vi "电流捕捉 v2.vi"(0 "task/channels in":refnum<k21> caption="任务/通道输入", 1 "触发后延时":u32=50, 2 "驱动值":dbl=10.0 format="%#_13g", 5 "条件":dbl=1.0, 7 "停止次数":i32=10, 11 "采样数":i32=500, 12 "CurrentType":enum16{"RMS均方根值", "AVG平均值"}(ring), 13 "停止值":dbl=1.0 format="%#_13g") -> (3 "输出波形":waveform(dbl), 4 "task out":refnum<k21>, 6 "最大电流":dbl format="%0.2f", 8 "电流值":dbl caption="均方根值" format="%.4f", 10 "能量":dbl, 15 "持续时间":dbl format="%0.2f")   [LabVIEW 2025]
uses:
  global.vi
  <vilib>/DAQmx/miscellaneous.llb/DAQmx Fill In Error Info.vi
  <vilib>/measure/NI_MAPro.lvlib
  <vilib>/Analysis/NI_AALBase.lvlib
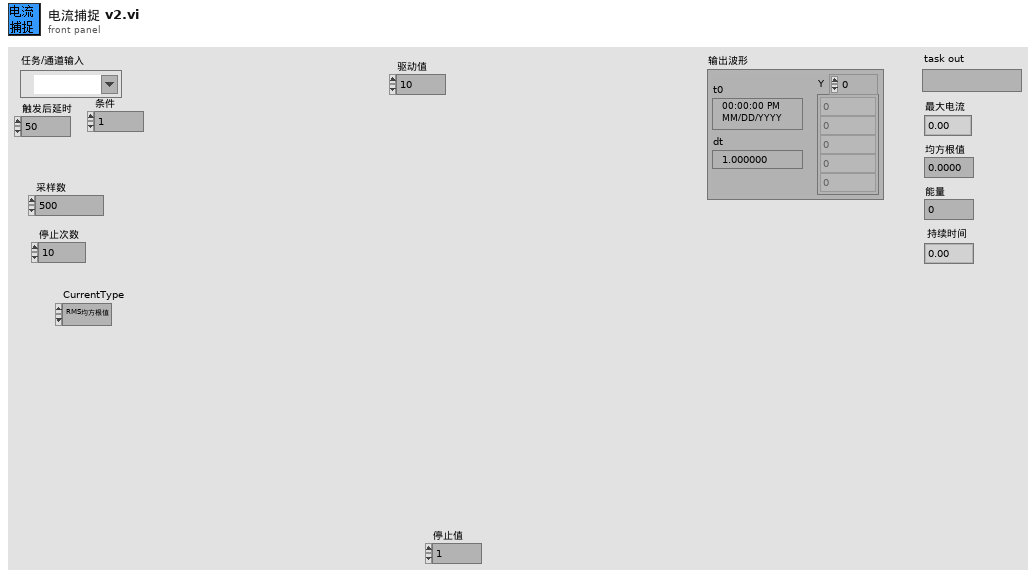
[diagram p1: front panel]
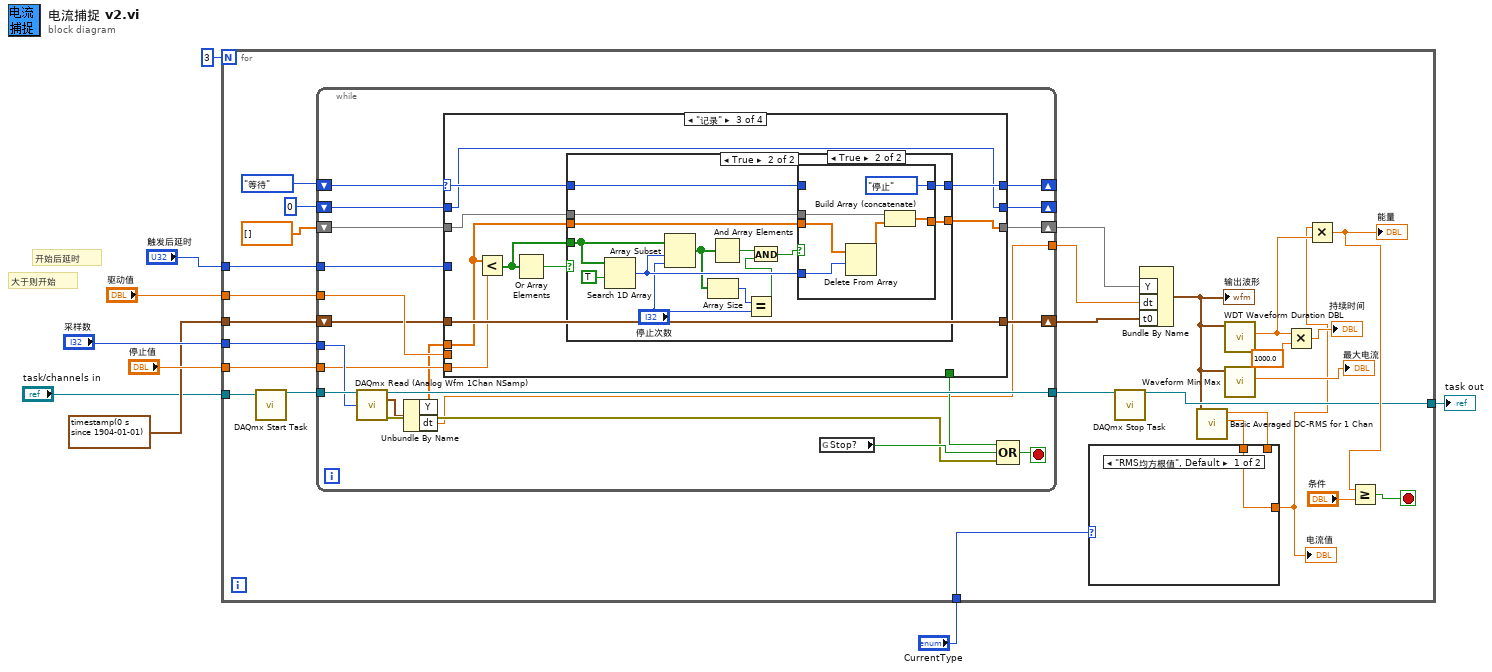
[diagram p0: block diagram]
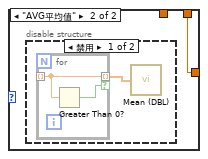
[diagram p2: hidden frame]
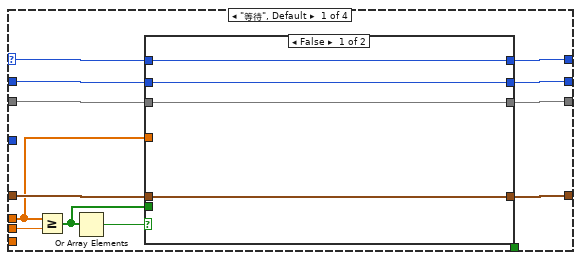
[diagram p4: hidden frame]
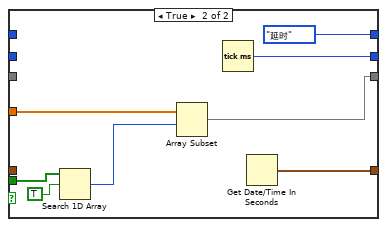
[diagram p5: hidden frame]
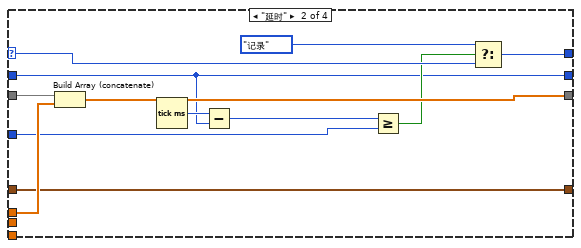
[diagram p6: hidden frame]
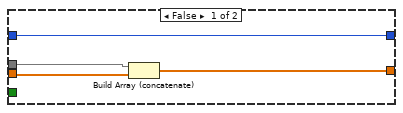
[diagram p7: hidden frame]
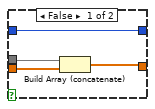
[diagram p8: hidden frame]
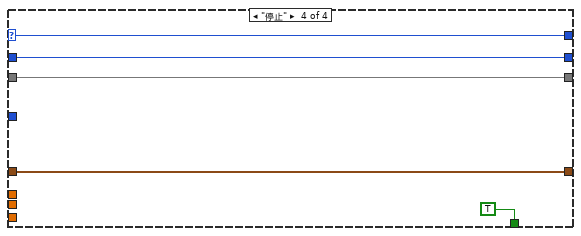
[diagram p9: hidden frame]
diagram:
  # "大于则开始"
  # "开始后延时"
  n1 = for {
    N: 3 -> [_]
    tunnel: "采样数" -> [w34]
    tunnel: "驱动值" -> [w33]
    tunnel: "触发后延时" -> [w30]
    tunnel: "停止值" -> [w29]
    tunnel: timestamp(0 s since 1904-01-01) -> [w27]
    tunnel: [w17] -> w2
    tunnel: "task/channels in" -> [w15]
    tunnel: "CurrentType" -> [w14]
    stop <- w23 stop-if-true
    n2 = call <vilib>:"DAQmx Start Task.vi"("task/channels in"=w15) -> ("task out"=w36:refnum<k21>)  [unwired: 13 in, 1 out]
    n3 = while {
      tunnel: w36 -> [w62]
      tunnel: w34 -> [w61]
      tunnel: [w60] -> w35
      shift-right: [w57] -> w24
      shift-left: dbl[] [] -> [w58]
      shift-right: [w56] -> _
      shift-left: enum16{"等待", "延时", "记录", "停止"}."等待" -> [w59]
      shift-right: [w51] -> _
      shift-left: u32 0 ("millisecond timer value") -> [w50]
      tunnel: w33 -> [w49]
      tunnel: w30 -> [w48]
      tunnel: w29 -> [w47]
      tunnel: [w42] -> w25
      shift-right: [w46] -> w28
      shift-left: w27 -> [w45]
      stop <- w55 stop-if-true
      n4 = call <vilib>:"DAQmx Read (Analog Wfm 1Chan NSamp).vi"("task/channels in"=w62, "number of samples per channel"=w61) -> ("task out"=w60:refnum<k21>, "data"=w44:waveform(dbl), "error out"=w52:errorcluster)  [unwired: 11 in]
      n5 = Unbundle By Name(w44) -> ("Y"=w43:dbl[], "dt"=w42:dbl)
      n6 = case shown="\"记录\"" w59 {
        selector: w59 -> [w71 w94 w108 w140]
        tunnel: w58 -> [w74 w98 w102 w141]
        tunnel: w43 -> [w65 w96 w104 _]
        tunnel: [w73 w97 w101 w141] -> w57
        tunnel: [w72 w95 w107 w140] -> w56
        tunnel: [_ _ _ TRUE] -> w54
        tunnel: [w70 w89 w106 w138] -> w51
        tunnel: w50 -> [w69 w89 w106 w138]
        tunnel: w49 -> [w68 _ _ _]
        tunnel: w48 -> [_ w88 _ _]
        tunnel: w47 -> [_ _ w100 _]
        tunnel: [w67 w87 w105 w137] -> w46
        tunnel: w45 -> [w66 w87 w105 w137]
        frame "等待", Default {
          n7 = Greater Or Equal?(x=w65, y=w68) -> (x >= y?=w63:bool[])
          n8 = Or Array Elements(Boolean array=w63) -> (logical OR=w64:bool)
          n9 = case shown="False" w64 {
            tunnel: w74 -> [w78 _]
            tunnel: w65 -> [_ w81]
            tunnel: [w78 w80] -> w73
            tunnel: [w77 enum16{"等待", "延时", "记录", "停止"}."延时"] -> w72
            tunnel: w71 -> [w77 _]
            tunnel: [w76 w85] -> w70
            tunnel: w69 -> [w76 _]
            tunnel: [w75 w84] -> w67
            tunnel: w66 -> [w75 _]
            tunnel: w63 -> [_ w83]
            frame False {
            }
            frame True {
              n10 = Search 1D Array(1D array=w83, element=TRUE) -> (index of element=w79:i32)  [unwired: 1 in]
              n11 = Array Subset(array=w81, index=w79) -> (w80:dbl[])  [unwired: 1 in]
              n12 = Tick Count (ms)() -> (millisecond timer value=w85:u32)
              n13 = Get Date/Time In Seconds() -> (seconds since 1Jan1904=w84:timestamp)
            }
          }
        }
        frame "延时" {
          n14 = Build Array (concatenate)(w98, w96) -> (w97:dbl[])
          n15 = Tick Count (ms)() -> (millisecond timer value=w91:u32)
          n16 = Subtract(x=w91, y=w89) -> (x-y=w90:u32)
          n17 = Greater Or Equal?(x=w90, y=w88) -> (x >= y?=w92:bool)
          n18 = Select(t=enum16{"等待", "延时", "记录", "停止"}."记录", s=w92, f=w94) -> (s? t:f=w95:enum16{"等待", "延时", "记录", "停止"})
        }
        frame "记录" {
          n19 = Less?(x=w104, y=w100) -> (x < y?=w99:bool[])
          n20 = Or Array Elements(Boolean array=w99) -> (logical OR=w103:bool)
          n21 = case shown="True" w103 {
            tunnel: w108 -> [w112 w119]
            tunnel: [w112 w126] -> w107
            tunnel: w104 -> [w111 w122]
            tunnel: w102 -> [w110 w125]
            tunnel: [w109 w124] -> w101
            tunnel: w99 -> [_ w123]
            frame False {
              n22 = Build Array (concatenate)(w110, w111) -> (w109:dbl[])
            }
            frame True {
              n23 = Search 1D Array(1D array=w123, element=TRUE ("元素")) -> (index of element=w120:i32)  [unwired: 1 in]
              n24 = Array Subset(array=w123, index=w120, length="停止次数") -> (w118:bool[])
              n25 = Array Size(array=w118) -> (size(s)=w117:i32)
              n26 = And Array Elements(Boolean array=w118) -> (logical AND=w115:bool)
              n27 = Equal?(x=w117, y="停止次数") -> (x = y?=w114:bool)
              n28 = And(x=w115, y=w114) -> (x .and. y?=w113:bool)
              n29 = case shown="True" w113 {
                tunnel: [w130 enum16{"等待", "延时", "记录", "停止"}."停止"] -> w126
                tunnel: w125 -> [w129 w135]
                tunnel: [w127 w134] -> w124
                tunnel: w122 -> [w128 w133]
                tunnel: w120 -> [_ w131]
                tunnel: w119 -> [w130 _]
                frame False {
                  n30 = Build Array (concatenate)(w129, w128) -> (w127:dbl[])
                }
                frame True {
                  n31 = Delete From Array(array=w133, length=w131) -> (array with subset deleted=w132:dbl[])  [unwired: 1 in, 1 out]
                  n32 = Build Array (concatenate)(w135, w132) -> (w134:dbl[])
                }
              }
            }
          }
        }
        frame "停止" {
        }
      }
      n33 = global read "global.vi" "Stop?"() -> (w53:bool)
      n34 = Compound Arithmetic op=OR(w54, w53, w52) -> (w55:bool)
    }
    n35 = call <vilib>:"DAQmx Stop Task.vi"("task/channels in"=w35) -> ("task out"=w17:refnum<k21>)  [unwired: 13 in, 1 out]
    n36 = Bundle By Name("Y"=w24, "dt"=w25, "t0"=w28) -> (w12:waveform(dbl))  [unwired: 1 in]
    "输出波形" <- w12
    n37 = call <vilib>:"Basic Averaged DC-RMS for 1 Chan.vi"("signal in"=w12) -> ("RMS value"=w10:dbl, "DC value"=w11:dbl)  [unwired: 7 in, 2 out]
    n38 = case shown="\"RMS均方根值\", Default" w14 {
      tunnel: [w37 w38] -> w13
      tunnel: w11 -> [_ w38]
      tunnel: w10 -> [w37 _]
      frame "RMS均方根值", Default {
      }
      frame "AVG平均值" {
        n39 = disable-structure shown="禁用" {
          frame Disabled {
            n40 = for {
              tunnel: _ -> [w41] mode=indexing
              tunnel: [w41] -> w39 mode=indexing if=w40
              n41 = Greater Than 0?(x=w41) -> (x > 0?=w40:bool)
            }
            n42 = call <vilib>:"Mean (DBL).vi"("X"=w39) -> ()  [unwired: 2 out]
          }
          frame Enabled {
          }
        }
      }
    }
    "电流值" <- w13
    n43 = call <vilib>:"WDT Waveform Duration DBL.vi"("waveform in"=w12) -> ("duration"=w16:dbl)  [unwired: 8 in, 2 out]
    n44 = call <vilib>:"Waveform Min Max.vi"("waveform in"=w12) -> ("Y max"=→"最大电流":dbl)  [unwired: 5 in, 5 out]
    n45 = Multiply(x=w16, y=1000.0) -> (x*y=→"持续时间":dbl)
    n46 = Multiply(x=w13, y=w16) -> (x*y=w22:dbl)
    "能量" <- w22
    n47 = Greater Or Equal?(x=w22, y="条件") -> (x >= y?=w23:bool)
  }
  "task out" <- w2
